vi "Start.vi"(8 "error in (no error)":errorcluster) -> (0 "error out":errorcluster)   [LabVIEW 2018, in "GLog.lvlib" / "Registry.lvlib"]
uses:
  Registry.lvlib
  Registry.vi
  Registry Global.vi
panel:
  # "Connector Pane"
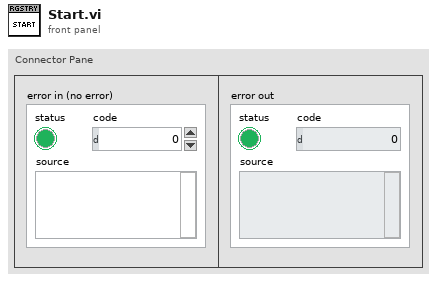
[diagram p1: front panel]
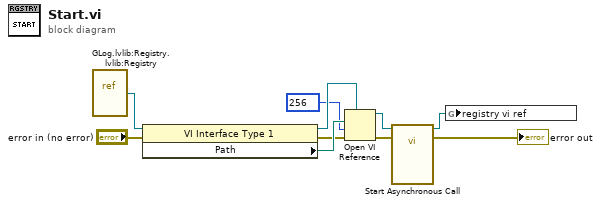
[diagram p0: block diagram]
diagram:
  n1 = vi-ref "GLog.lvlib:Registry.lvlib:Registry.vi"() -> (w9:refnum<vi>)
  n2 = property class="VI Interface Type 1"(reference=w9, error in="error in (no error)") -> (reference out=w8:refnum<vi>, error out=w4:errorcluster, "Path"=w10:path)
  n3 = Open VI Reference(type specifier VI Refnum (for type only)=w8, vi path=w10, options=256, error in (no error)=w4) -> (vi reference=w3:refnum<vi>, error out=w5:errorcluster)  [unwired: 2 in]
  n4 = call-by-ref "Start Asynchronous Call"(reference=w3, error in=w5) -> (reference out=w1:refnum<vi>, error out=→"error out":errorcluster)  [unwired: 12 in]
  n5 = global write "Registry Global.vi" "registry vi ref"(w1) -> ()
